vi "Add Copyright to Folder.vi"(8 "error in (no error)":errorcluster, 9 "Type":T1={"vi"=TRUE, "ctl"=TRUE, "lvlib"=TRUE, "lvclass"=TRUE, "lvproj"=TRUE} caption="Select File Type to Add Copyright", 10 "Copyright Text":string="© Company Name", 11 "Source Code Directory":path) -> (0 "error out":errorcluster)   [LabVIEW 2016, in "SLL Add Copyright.lvlib"]
doc: "Add/update copyright text to all LabVIEW files in the provided folder. \n\nSupported LabVIEW files are *.vi, *.ctl, *.lvlib, *.lvclass and *.lvproj."
uses:
  SLL Add Copyright.lvlib
  _Typedefs/Select File Type.ctl
panel:
  out "Progress":i32(slide) scale=0.0..5.0
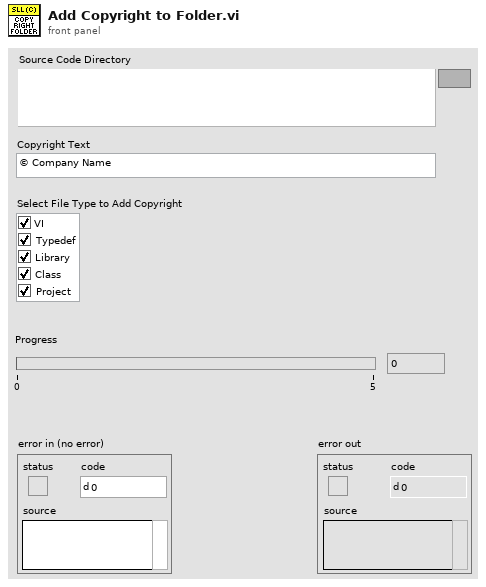
[diagram p1: front panel]
types:
  T1 = typedef "SLL Add Copyright.lvlib/Select File Type.ctl" = cluster{"vi":bool, "ctl":bool, "lvlib":bool, "lvclass":bool, "lvproj":bool}
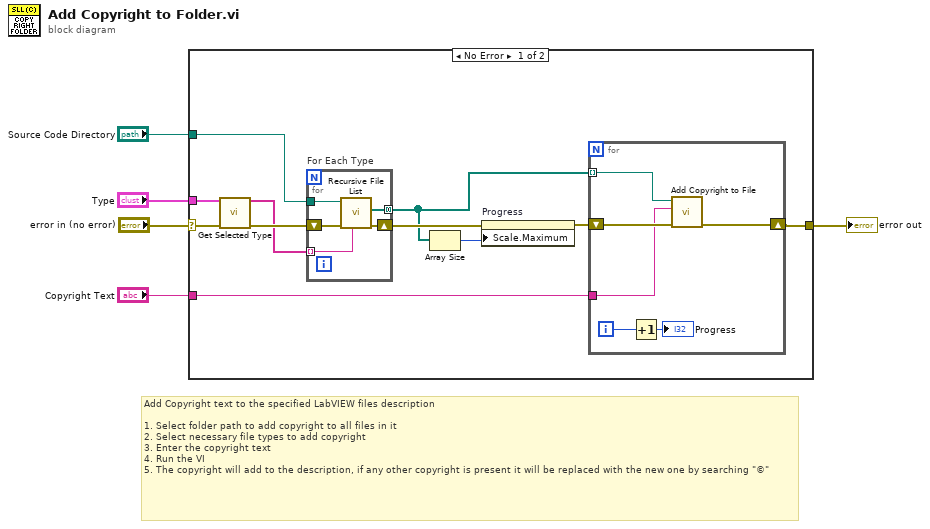
[diagram p0: block diagram]
diagram:
  # "Add Copyright text to the specified LabVIEW files description\n\n1. Select folder path to add copyright to all files in it\n2. Select necessary file types to add copyright\n3. Enter the copyright text\n4. Run the VI\n5. The copyright will add to the description, if any other copyright is present it will be replaced with the new one by searching \"©\""
  n1 = case shown="No Error" "error in (no error)" {
    selector: "error in (no error)" -> [w6 w28]
    tunnel: "Type" -> [w16 _]
    tunnel: "Source Code Directory" -> [w12 _]
    tunnel: "Copyright Text" -> [w8 _]
    tunnel: [w7 w28] -> w2
    frame No Error {
      n2 = call "Get Selected Type.vi"("Select Type"=w16, "error in (no error)"=w6) -> ("Selected File Types[]"=w11:string[], "error out"=w14:errorcluster)  [unwired: 12 in]
      n3 = for "For Each Type" {
        tunnel: w12 -> [w19]
        tunnel: w11 -> [w18] mode=indexing
        tunnel: [w17] -> w10 mode=concatenating
        shift-right: [w20] -> w13
        shift-left: w14 -> [w21]
        n4 = call <vilib>:"Recursive File List.vi"("pattern"=w18, "error in (no error)"=w21, "Folder Path"=w19) -> ("error out"=w20:errorcluster, "All Files in Dir"=w17:path[])  [unwired: 4 in, 3 out]
      }
      n5 = Array Size(array=w10) -> (size(s)=w9:i32)
      n6 = property on="Progress" class="Slide (strict)"(error in=w13, "Scale.Maximum"=w9) -> (error out=w15:errorcluster)  [unwired: 1 in, 1 out]
      n7 = for {
        shift-right: [w25] -> w7
        shift-left: w15 -> [w26]
        tunnel: w10 -> [w27] mode=indexing
        tunnel: w8 -> [w22]
        i -> [w24]
        n8 = Increment(x=w24) -> (x+1=→"Progress":i32)
        n9 = call "Add Copyright to File.vi"("error in (no error)"=w26, "Copyright Text"=w22, "File Path"=w27) -> ("error out"=w25:errorcluster)  [unwired: 8 in]
      }
    }
    frame Error {
    }
  }
  "error out" <- w2
